vi "Error Handler.vi"(8 "error in (no error)":errorcluster, 11 "queue":refnum<queue>) -> (0 "error out":errorcluster, 3 "Errors":string)   [LabVIEW 2021]
uses:
  Type defs/Message cluster.ctl
  Type defs/Error FGV States.ctl
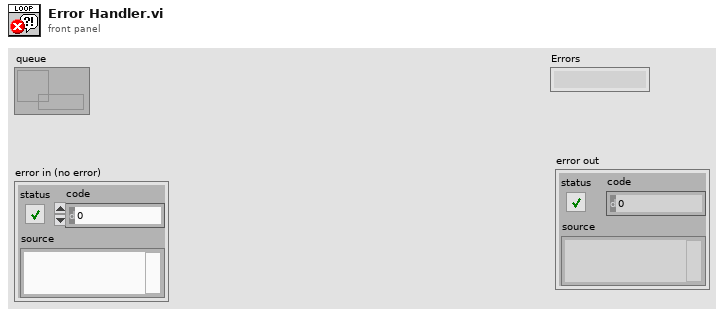
[diagram p1: front panel]
types:
  T1 = typedef "Error FGV States.ctl" = enum16{"Save", "Clear", "Add", "Read"}
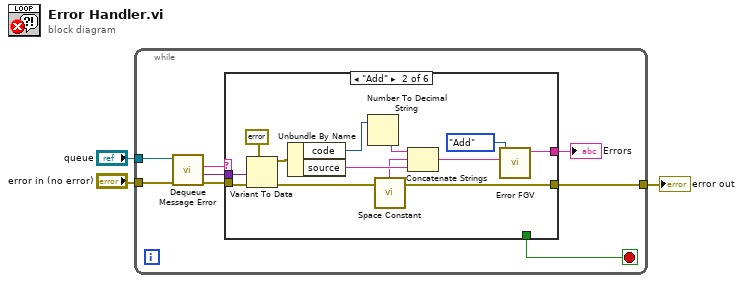
[diagram p0: block diagram]
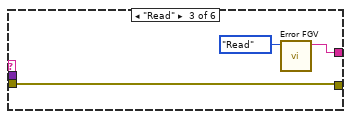
[diagram p3: hidden frame]
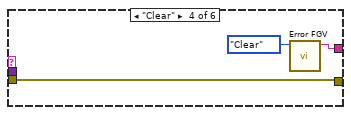
[diagram p4: hidden frame]
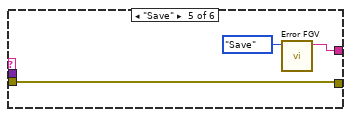
[diagram p5: hidden frame]
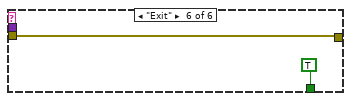
[diagram p6: hidden frame]
diagram:
  n1 = while {
    tunnel: "queue" -> [w10]
    tunnel: "error in (no error)" -> [w9]
    tunnel: [w4] -> w1
    stop <- w5 stop-if-true
    n2 = call "Dequeue Message Error.vi"("error in (no error)"=w9, "Message Queue"=w10) -> ("error out"=w7:errorcluster, "Data"=w8:variant, "Message"=w11:string)  [unwired: 6 in, 1 out]
    n3 = case shown="\"Add\"" w11 {
      tunnel: w8 -> [_ w22 _ _ _ _]
      tunnel: w7 -> [_ w23 w26 w29 w32 w33]
      tunnel: [_ w14 w26 w29 w32 w33] -> w4
      tunnel: [_ w13 w25 w28 w31 _] -> w6
      tunnel: [_ _ _ _ _ TRUE] -> w5
      frame Default {
      }
      frame "Add" {
        n4 = Variant To Data(error in=w23, type=errorcluster {"status"=FALSE, "code"=0, "source"=""} ("error in (no error)"), Variant=w22) -> (data=w20:errorcluster, error out=w14:errorcluster)
        n5 = Unbundle By Name(w20) -> ("code"=w12:i32, "source"=w18:string)
        n6 = Number To Decimal String(number=w12) -> (decimal integer string=w19:string)  [unwired: 1 in]
        n7 = call <vilib>:"Space Constant.vi"() -> ("String"=w17:string)
        n8 = Concatenate Strings(w19, w17, w18) -> (w16:string)
        n9 = call "Error FGV.vi"("New Error"=w16, "FGV states"=Error_FGV_States."Add") -> ("Errors"=w13:string)  [unwired: 9 in]
      }
      frame "Read" {
        n10 = call "Error FGV.vi"("FGV states"=Error_FGV_States."Read") -> ("Errors"=w25:string)  [unwired: 10 in]
      }
      frame "Clear" {
        n11 = call "Error FGV.vi"("FGV states"=Error_FGV_States."Clear") -> ("Errors"=w28:string)  [unwired: 10 in]
      }
      frame "Save" {
        n12 = call "Error FGV.vi"("FGV states"=Error_FGV_States."Save") -> ("Errors"=w31:string)  [unwired: 10 in]
      }
      frame "Exit" {
      }
    }
    "Errors" <- w6
  }
  "error out" <- w1
